vi "getVideo.vi"(8 "error in (no error)":errorcluster, 10 "Video Id":string, 11 "YoutubeCacheProxy in":refnum<class "YoutubeCacheProxy.lvclass">) -> (0 "error out":errorcluster, 2 "Video":refnum<class "Video.lvclass">, 3 "YoutubeCacheProxy out":refnum<class "YoutubeCacheProxy.lvclass">)   [LabVIEW 2018, in "YoutubeCacheProxy.lvclass"]
uses:
  YoutubeCacheProxy.lvclass
  Video Class/Video.lvclass
  YoutubeCacheProxy.lvclass/YoutubeCacheProxy.ctl
  ConsoleOut/Print Options.ctl
  ThirdPartyYoutubeLib Class/ThirdPartyYoutubeLib.lvclass
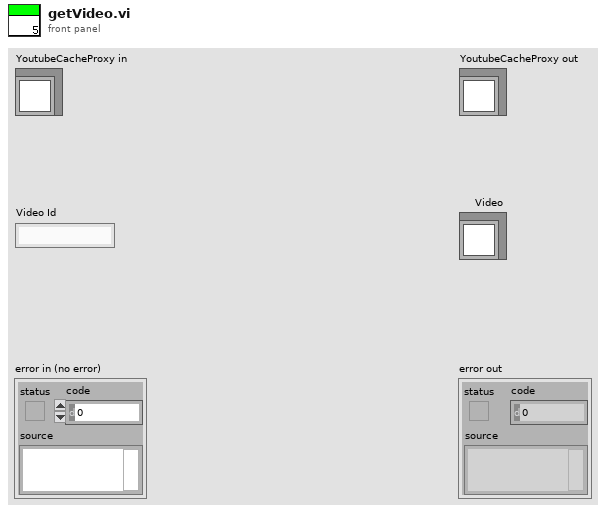
[diagram p1: front panel]
types:
  T1 = typedef "Print Options.ctl" = enum16{"Create", "Get Reference", "Print", "Print Header", "Close"}
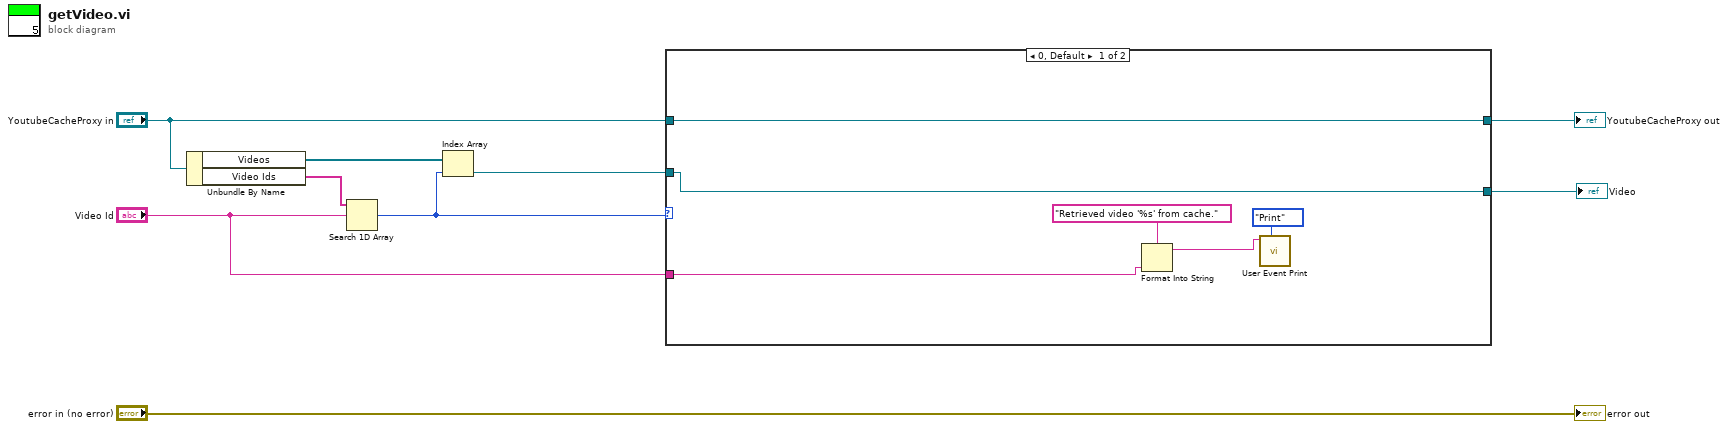
[diagram p0: block diagram]
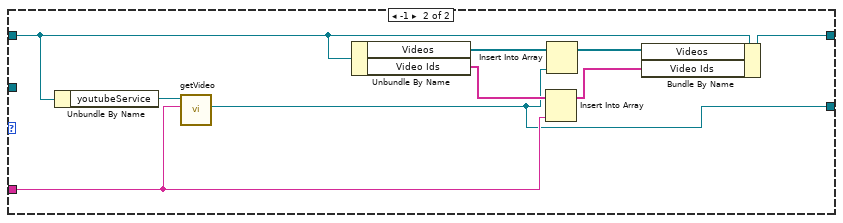
[diagram p2: hidden frame]
diagram:
  n1 = Unbundle By Name("YoutubeCacheProxy in") -> ("Videos"=w2:refnum<class "Video.lvclass">[], "Video Ids"=w8:string[])
  n2 = Search 1D Array(1D array=w8, element="Video Id") -> (index of element=w1:i32)  [unwired: 1 in]
  n3 = Index Array(array=w2, index=w1) -> (element=w3:refnum<class "Video.lvclass">)
  n4 = case shown="0, Default" w1 {
    tunnel: "YoutubeCacheProxy in" -> [w15 w22]
    tunnel: [w15 w23] -> w6
    tunnel: "Video Id" -> [w12 w17]
    tunnel: [w14 w16] -> w4
    tunnel: w3 -> [w14 _]
    frame 0, Default {
      n5 = Format Into String(format string="Retrieved video '%s' from cache.", w12) -> (resulting string=w11:string)  [unwired: 2 in, 1 out]
      n6 = call "User Event Print.vi"("Options"=Print_Options."Print", "String to Print"=w11) -> ()  [unwired: 8 in, 2 out]
    }
    frame -1 {
      n7 = Unbundle By Name(w22) -> ("youtubeService"=w24:refnum<class "ThirdPartyYoutubeLib.lvclass">)
      n8 = call-dynamic "getVideo.vi"("Video Id"=w17, "ThirdPartyYoutubeLib in"=w24) -> ("Video"=w16:refnum<class "Video.lvclass">)  [unwired: 7 in, 2 out]
      n9 = Unbundle By Name(w22) -> ("Videos"=w21:refnum<class "Video.lvclass">[], "Video Ids"=w19:string[])
      n10 = Insert Into Array(array=w19, new element=w17) -> (w18:string[])  [unwired: 1 in]
      n11 = Insert Into Array(array=w21, new element=w16) -> (w20:refnum<class "Video.lvclass">[])  [unwired: 1 in]
      n12 = Bundle By Name(cluster=w22, "Videos"=w20, "Video Ids"=w18) -> (w23:refnum<class "YoutubeCacheProxy.lvclass">)
    }
  }
  "YoutubeCacheProxy out" <- w6
  "Video" <- w4
  "error out" <- "error in (no error)"
